vi "Generate Library Icon.vi"(8 "error in (no error)":errorcluster, 11 "Library Refnum in":refnum<vi>) -> (0 "error out":errorcluster, 3 "Library Refnum out":refnum<vi>)   [LabVIEW 2020, in "Project Provider.lvlib"]
uses:
  Project Provider.lvlib
  <vilib>/LabVIEW Icon API/lv_icon/classes/Icon/Icon.lvclass
  <vilib>/LabVIEW Icon API/API_Rectangle Dimension.ctl
  <vilib>/LabVIEW Icon API/API_Text.ctl
  <vilib>/LabVIEW Icon API/API_Rectangle Colors.ctl
  <vilib>/LabVIEW Icon API/LabVIEW Icon API.lvlib
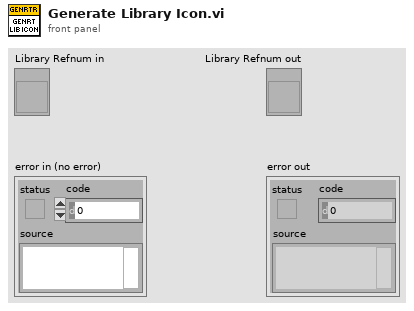
[diagram p1: front panel]
types:
  T1 = typedef "LabVIEW Icon API.lvlib/API_Rectangle Colors.ctl" = cluster{"Border":u32, "Background":u32}
  T2 = typedef "LabVIEW Icon API.lvlib/API_Text.ctl" = cluster{"Line 1 text":string, "Line 2 text":string, "Line 3 text":string, "Line 4 text":string}
  T3 = typedef "LabVIEW Icon API.lvlib/API_Rectangle Dimension.ctl" = cluster{"Width":i16, "Height":i16}
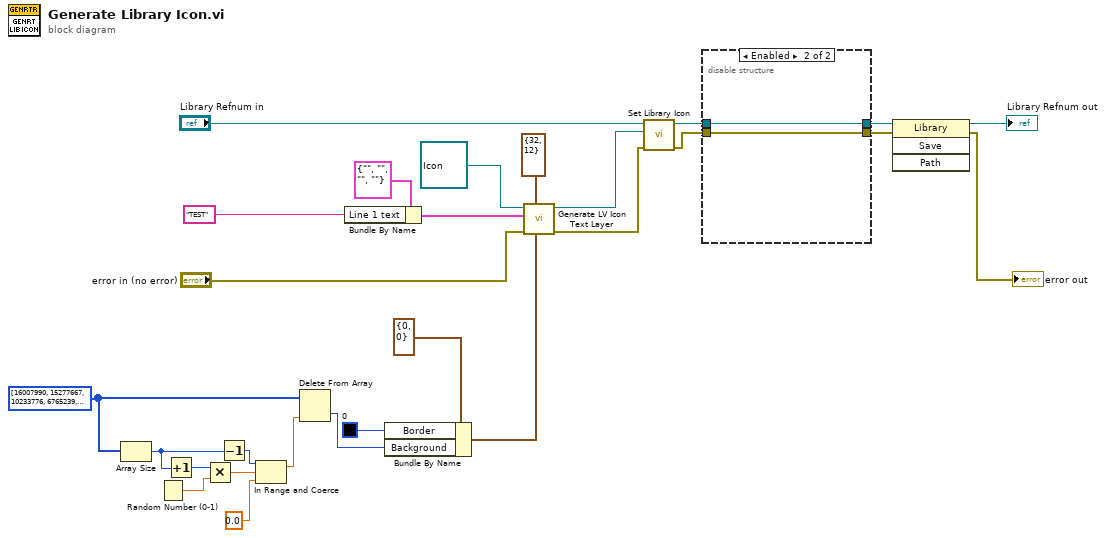
[diagram p0: block diagram]
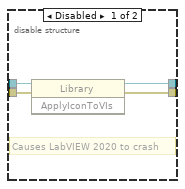
[diagram p2: hidden frame]
diagram:
  w15 = u32[] [16007990, 15277667, 10233776, 6765239, 4149685, 2201331, 240116, 48340, 38536, 5025616, 9159498, 13491257, 16771899, 16761095, 16750592, 16733986, 7951688, 10395294, 6323595] ("Array")
  n1 = Array Size(array=w15) -> (size(s)=w9:i32)
  n2 = Random Number (0-1)() -> (number: 0 to 1=w8:dbl)
  n3 = Increment(x=w9) -> (x+1=w10:i32)
  n4 = Multiply(x=w10, y=w8) -> (x*y=w13:dbl)
  n5 = Decrement(x=w9) -> (x-1=w12:i32)
  n6 = In Range and Coerce(upper limit=w12, x=w13, lower limit=0.0) -> (coerced(x)=w7:dbl)  [unwired: 1 out]
  n7 = Delete From Array(array=w15, index=w7) -> (deleted portion=w14:u32)  [unwired: 1 in, 1 out]
  n8 = Bundle By Name(cluster=T2 {"Line 1 text"="", "Line 2 text"="", "Line 3 text"="", "Line 4 text"=""} ("Text"), "Line 1 text"="TEST" ("Overlay Text")) -> (w23:T2)
  n9 = Bundle By Name(cluster=T1 {"Border"=0, "Background"=0} ("Library Color"), "Border"=u32 0 ("Background"), "Background"=w14) -> (w16:T1)
  n10 = call <vilib>:"Generate LV Icon Text Layer.vi"("Rectangle colors (black, white)"=w16, "Rectangle dimension (32,32)"=T3 {"Width"=32, "Height"=12}, "error in (no error)"="error in (no error)", "Text"=w23, "Icon in"=refnum<class "Icon.lvclass"> refnum ("Icon.lvclass in")) -> ("error out"=w20:errorcluster, "Icon out"=w24:refnum<class "Icon.lvclass">)  [unwired: 5 in]
  n11 = call <vilib>:"Set Library Icon.vi"("error in (no error)"=w20, "Icon"=w24, "Library Refnum in"="Library Refnum in") -> ("error out"=w19:errorcluster, "Library Refnum out"=w2:refnum<vi>)  [unwired: 7 in]
  n12 = disable-structure shown="Enabled" {
    disable-tunnel: w19 -> [w31 w32]
    disable-tunnel: [w30 w32] -> w3
    disable-tunnel: w2 -> [w29 w33]
    disable-tunnel: [w28 w33] -> w1
    frame Disabled {
      # "Causes LabVIEW 2020 to crash"
      n13 = invoke class="Library" method="ApplyIconToVIs"(reference=w29, error in=w31) -> (reference out=w28:refnum<vi>, error out=w30:errorcluster)  [unwired: 1 in, 1 out]
    }
    frame Enabled {
    }
  }
  n14 = invoke class="Library" method="Save"(reference=w1, error in=w3) -> (reference out=→"Library Refnum out":refnum<vi>, error out=→"error out":errorcluster)  [unwired: 2 in, 2 out]
